vi "F to C convertor.vi"(8 "Temp(F) 4":dbl, 9 "Temp(F) 3":dbl, 10 "Temp(F) 2":dbl, 11 "Temp(F)":dbl) -> (0 "Temp (C) 4":dbl, 1 "Temp (C) 3":dbl, 2 "Temp (C) 2":dbl, 3 "Temp (C)":dbl)   [LabVIEW 2025]
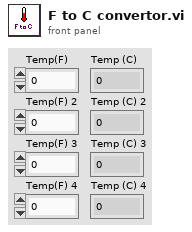
[diagram p1: front panel]
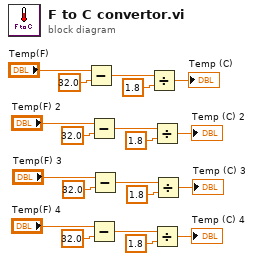
[diagram p0: block diagram]
diagram:
  n1 = Subtract(x="Temp(F)", y=32.0) -> (x-y=w18:dbl)
  n2 = Subtract(x="Temp(F) 2", y=32.0) -> (x-y=w13:dbl)
  n3 = Subtract(x="Temp(F) 4", y=32.0) -> (x-y=w3:dbl)
  n4 = Subtract(x="Temp(F) 3", y=32.0) -> (x-y=w8:dbl)
  n5 = Divide(x=w18, y=1.8) -> (x/y=→"Temp (C)":dbl)
  n6 = Divide(x=w13, y=1.8) -> (x/y=→"Temp (C) 2":dbl)
  n7 = Divide(x=w3, y=1.8) -> (x/y=→"Temp (C) 4":dbl)
  n8 = Divide(x=w8, y=1.8) -> (x/y=→"Temp (C) 3":dbl)
